vi "Create_Analog_Pair.vi"(7 "section":string, 8 "error in (no error)":errorcluster, 9 "Analog Pair Key":T1={"AI_Channel"="Speed_AI_Channel", "AO_Channel"="AO_Channel"}, 10 "Modbus_Master.lvclass":refnum<class "Modbus_Master.lvclass">, 11 "Config File in":path) -> (0 "error out":errorcluster, 1 "AnalogInput.lvclass":refnum<class "AnalogInput.lvclass">, 2 "AnalogOutput.lvclass":refnum<class "AnalogOutput.lvclass">, 3 "Config File Out":path)   [LabVIEW 2021]
uses:
  AnalogOutput/AnalogOutput.lvclass
  AnalogInput/AnalogInput.lvclass
  Modbus_Master/Modbus_Master.lvclass
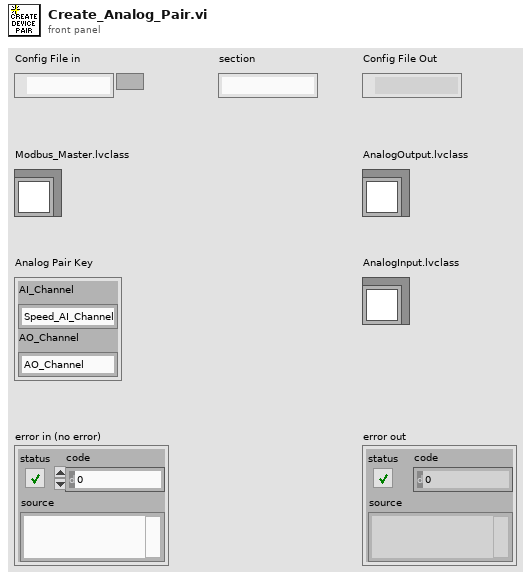
[diagram p1: front panel]
types:
  T1 = cluster{"AI_Channel":string, "AO_Channel":string}
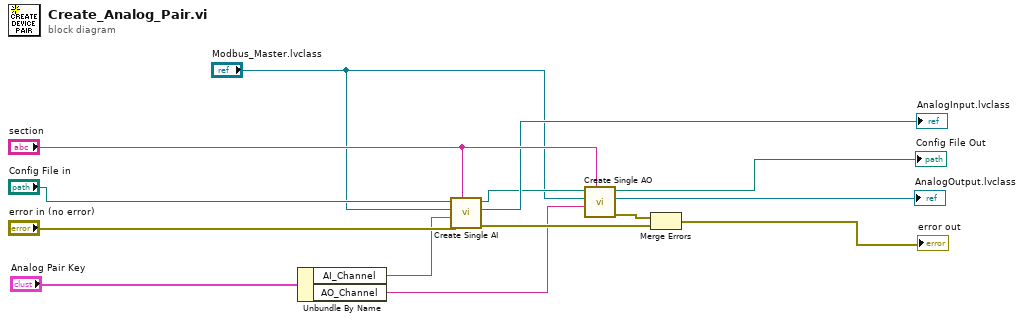
[diagram p0: block diagram]
diagram:
  n1 = Unbundle By Name("Analog Pair Key") -> ("AI_Channel"=w3:string, "AO_Channel"=w2:string)
  n2 = call "Create Single AI.vi"("section"="section", "error in (no error)"="error in (no error)", "AI_Channel"=w3, "Modbus_Master.lvclass"="Modbus_Master.lvclass", "Path In"="Config File in") -> ("error out"=w6:errorcluster, "AnalogInput.lvclass"=→"AnalogInput.lvclass":refnum<class "AnalogInput.lvclass">, "Path Out"=w4:path)  [unwired: 4 in]
  n3 = call "Create Single AO.vi"("section"="section", "AO_Channel"=w2, "Modbus_Master.lvclass"="Modbus_Master.lvclass", "Config File In"=w4) -> ("error out"=w5:errorcluster, "AnalogOutput.lvclass"=→"AnalogOutput.lvclass":refnum<class "AnalogOutput.lvclass">, "Config File Out"=→"Config File Out":path)  [unwired: 5 in]
  n4 = Merge Errors(w5, w6) -> (→"error out":errorcluster)
